vi "Create Response-JSONtext.vi"(6 "id":string, 8 "error in (no error)":errorcluster, 10 "result":variant) -> (0 "error out":errorcluster, 2 "<JSON>":string="{\"jsonrpc\":\"2.0\",\"id\":\"\"}")   [LabVIEW 2019, in "JSON-RPC.lvlib"]
uses:
  JSON-RPC.lvlib
  8844cadd-62f3-4521-a403-8b9f5f002626.vi
  <vilib>/JDP Science/JSONtext/Variant to JSON Text.vi
  <vilib>/JDP Science/JSONtext/LVClass Serializer/JSONtext LVClass Serializer.lvclass
  <vilib>/JDP Science/JSONtext/JSONtext.lvlib
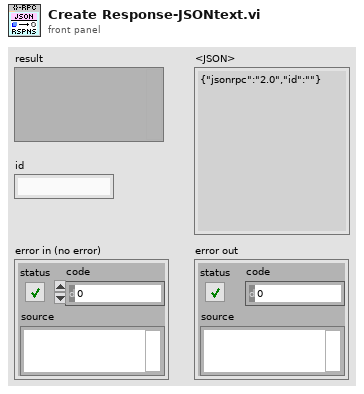
[diagram p1: front panel]
types:
  T1 = typedef "JSON-RPC.lvlib/Error--Cluster.ctl" = cluster{"code":i32, "message":string}
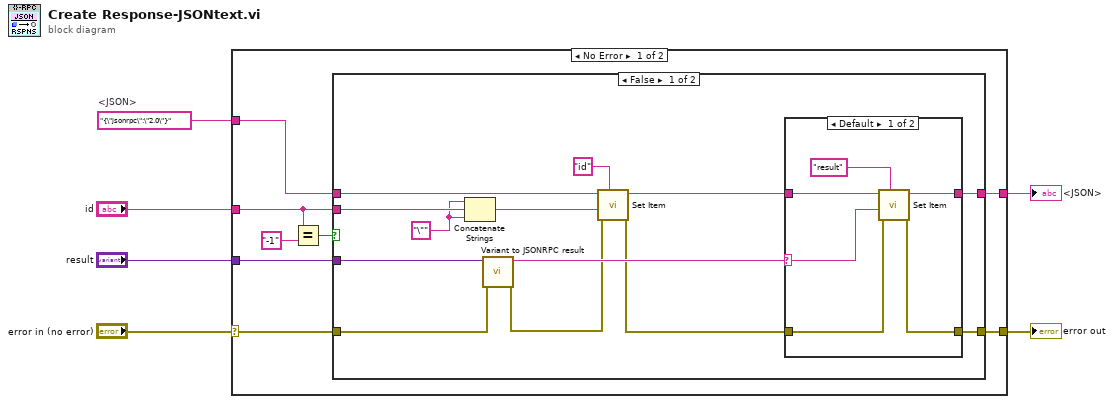
[diagram p0: block diagram]
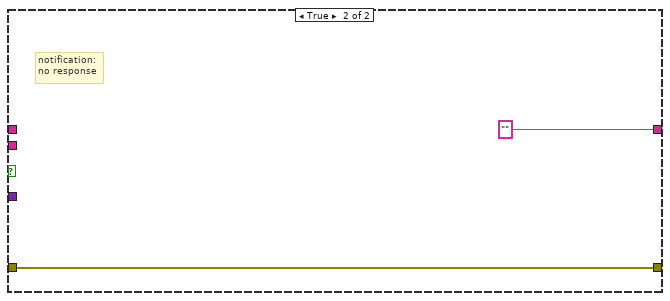
[diagram p3: hidden frame]
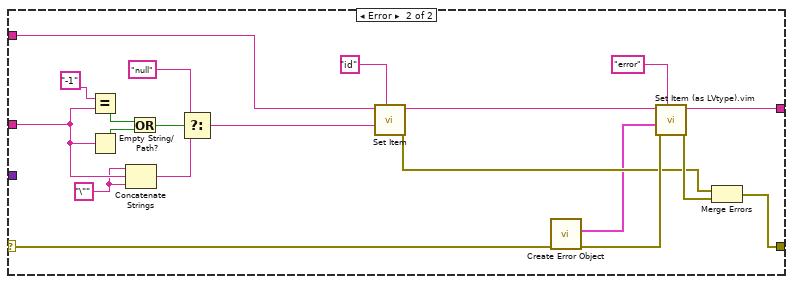
[diagram p4: hidden frame]
diagram:
  w1 = "{\"jsonrpc\":\"2.0\"}"  # <JSON>
  n1 = case shown="No Error" "error in (no error)" {
    selector: "error in (no error)" -> [w13 w47]
    tunnel: [w11 w39] -> w6
    tunnel: [w12 w50] -> w5
    tunnel: "id" -> [w8 w43]
    tunnel: "result" -> [w14 _]
    tunnel: w1 -> [w9 w45]
    frame No Error {
      n2 = Equal?(x=w8, y="-1" ("x")) -> (x = y?=w10:bool)
      n3 = case shown="False" w10 {
        tunnel: w14 -> [w27 _]
        tunnel: w13 -> [w26 w36]
        tunnel: [w19 "" ("<JSON>")] -> w12
        tunnel: w8 -> [w18 _]
        tunnel: [w21 w36] -> w11
        tunnel: w9 -> [w17 _]
        frame False {
          w15 = "\"" ("string")
          n4 = Concatenate Strings(w15, w18, w15) -> (w16:string)
          n5 = call "Variant to JSONRPC result .vi"("error in (no error)"=w26, "variant"=w27) -> ("error out"=w23:errorcluster, "<JSON>"=w25:string)  [unwired: 8 in]
          n6 = call <vilib>:"Set Item.vi"("$Path or Item Name"="id", "error in (no error)"=w23, "JSON to Insert"=w16, "JSON"=w17) -> ("error out"=w22:errorcluster, "<JSON>"=w20:string)  [unwired: 4 in, 1 out]
          n7 = case shown="Default" w25 {
            selector: w25 -> [w28 _]
            tunnel: w22 -> [w31 w35]
            tunnel: [w32 w35] -> w21
            tunnel: w20 -> [w30 w34]
            tunnel: [w29 w34] -> w19
            frame Default {
              n8 = call <vilib>:"Set Item.vi"("$Path or Item Name"="result" ("String"), "error in (no error)"=w31, "JSON to Insert"=w28, "JSON"=w30) -> ("error out"=w32:errorcluster, "<JSON>"=w29:string)  [unwired: 4 in, 1 out]
            }
            frame "null" {
            }
          }
        }
        frame True {
          # "notification:\nno response"
        }
      }
    }
    frame Error {
      w42 = "\"" ("string")
      n9 = Equal?(x="-1" ("y"), y=w43) -> (x = y?=w57:bool)
      n10 = Empty String/Path?(string/path=w43) -> (empty?=w56:bool)
      n11 = Concatenate Strings(w42, w43, w42) -> (w41:string)
      n12 = Or(x=w57, y=w56) -> (x .or. y?=w55:bool)
      n13 = Select(t="null", s=w55, f=w41) -> (s? t:f=w44:string)
      n14 = call <vilib>:"Set Item.vi"("$Path or Item Name"="id", "JSON to Insert"=w44, "JSON"=w45) -> ("error out"=w40:errorcluster, "<JSON>"=w48:string)  [unwired: 5 in, 1 out]
      n15 = call "Create Error Object.vi"("error in (no error)"=w47) -> ("error out"=w52:errorcluster, "error"=w38:T1)  [unwired: 9 in]
      n16 = call "Set Item (as LVtype).vim"("$Path or Item Name"="error", "error in (no error)"=w52, "Anything"=w38, "JSON"=w48) -> ("error out"=w46:errorcluster, "<JSON>"=w50:string)  [unwired: 4 in, 1 out]
      n17 = Merge Errors(w40, w46) -> (w39:errorcluster)
    }
  }
  "error out" <- w6
  "<JSON>" <- w5
